vi "Request State Store.vi"(5 "arguments digest":string, 6 "name":string, 7 "method":string, 8 "error in":errorcluster, 9 "state":string, 10 "token":string, 11 "action":enum16{"store", "take", "clear"}(ring)) -> (0 "error out":errorcluster, 1 "entry":T1, 2 "found?":bool, 3 "new token":string)   [LabVIEW 2020, in "MCP Server.lvlib"]
doc: "Keeps the server-side state of multi round-trip requests (MCP 2026-07-28, requestState) and hands out the opaque tokens that stand for it. A functional global: the entries live in uninitialized shift registers of this non-reentrant VI, so every caller in the application instance sees the same store.\n\nWHY: a tool that asks several questions in several rounds (Ask User.vi) needs the answers of the earlier rounds, but the client sends back only the answers to the latest inputRequests. So the server keeps the earlier answers here and gives the client only a random token as requestState. The client never holds content it could tamper with; an unknown, expired or mis-bound token is simply not found.\n\naction:\n- store: keeps {token, state, method, name, arguments digest, created} and returns the new token. The token is \"mcp-rs-\" followed by 32 hex characters, the first half (16 bytes) of the SHA-256 (SHA-256 Byte Array Checksum.vi of NI's Message Digest API) of four random numbers, the tick count, a running counter and the state text.\n- take: looks the token up. found? is TRUE and entry holds the stored entry when it is known and not expired. Entries are NOT removed by take: a client may legitimately send the same round again after a network failure.\n- clear: forgets every entry.\n\nEvery call first drops the entries older than 10 minutes (600000 ms by Tick Count), and store keeps at most the 64 newest entries.\n\nUsed by Resolve Request State.vi (take) and Input Required Response.vi (store). error in is passed through unchanged; the store works whatever error in carries, and has no errors of its own."
uses:
  MCP Server.lvlib
  <vilib>/security/Message Digest/API/NI_Message Digest API.lvlib
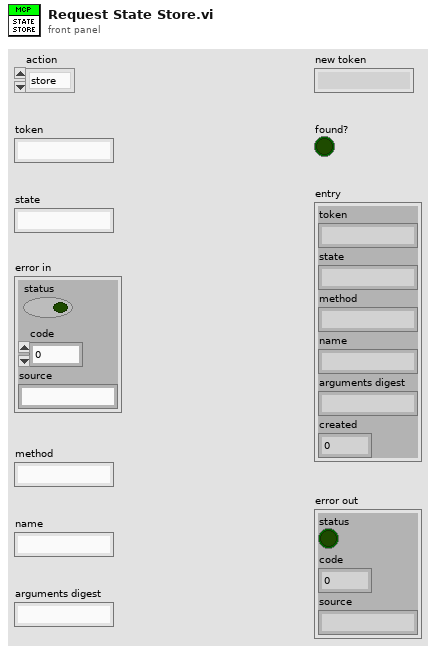
[diagram p1: front panel]
types:
  T1 = cluster{"token":string, "state":string, "method":string, "name":string, "arguments digest":string, "created":u32}
  T2 = cluster{"token":string, "state":string, "method":string, "name":string, "arguments digest":string, "created":u32}[]
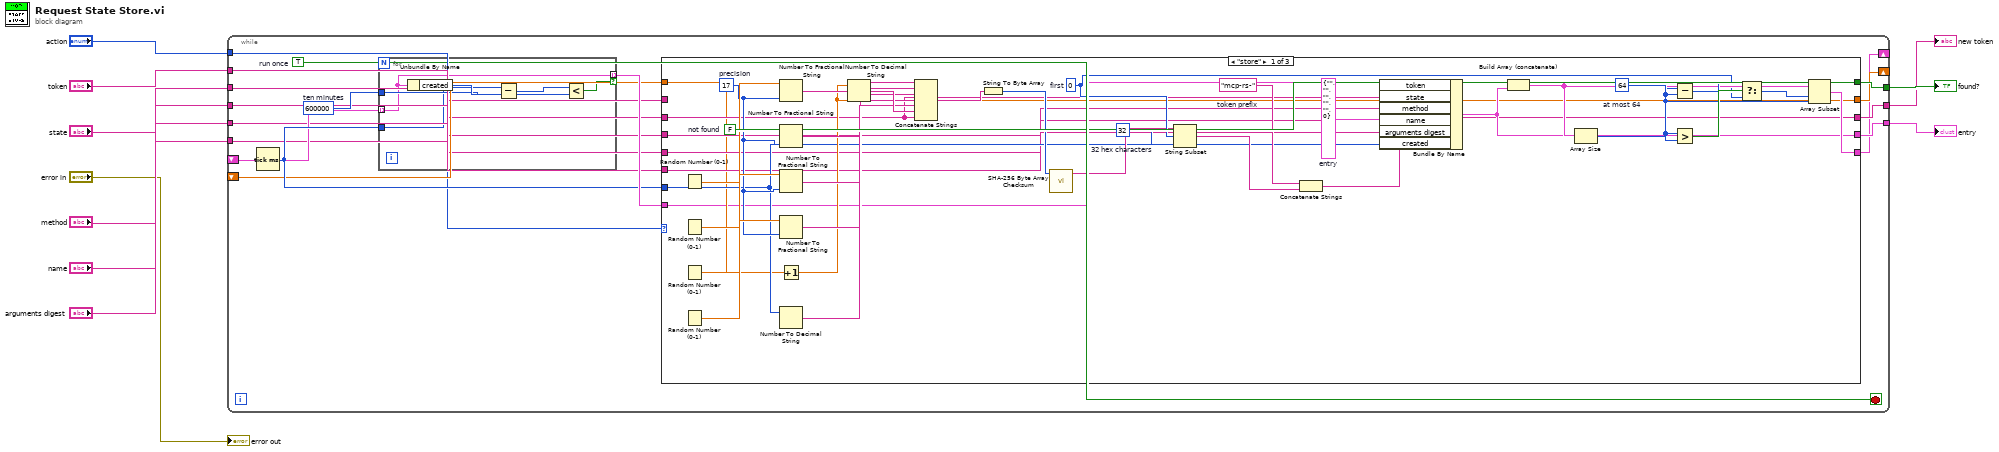
[diagram p0: block diagram]
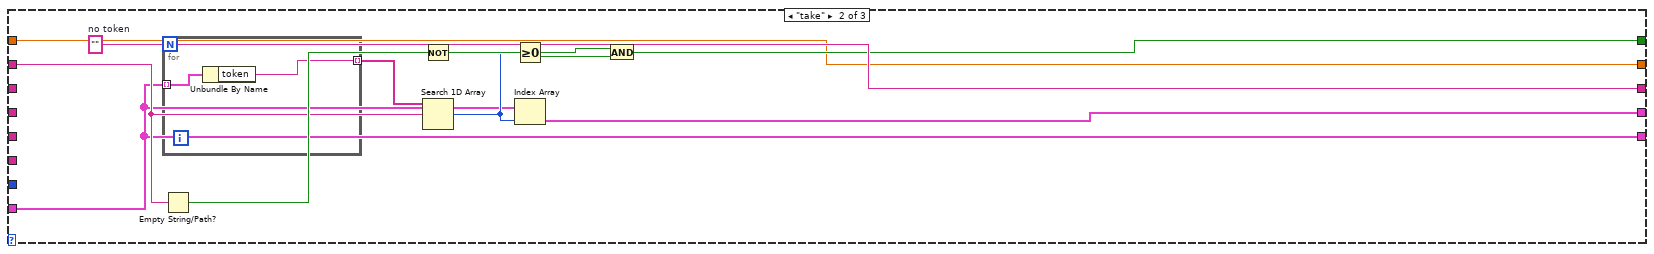
[diagram p2: hidden frame]
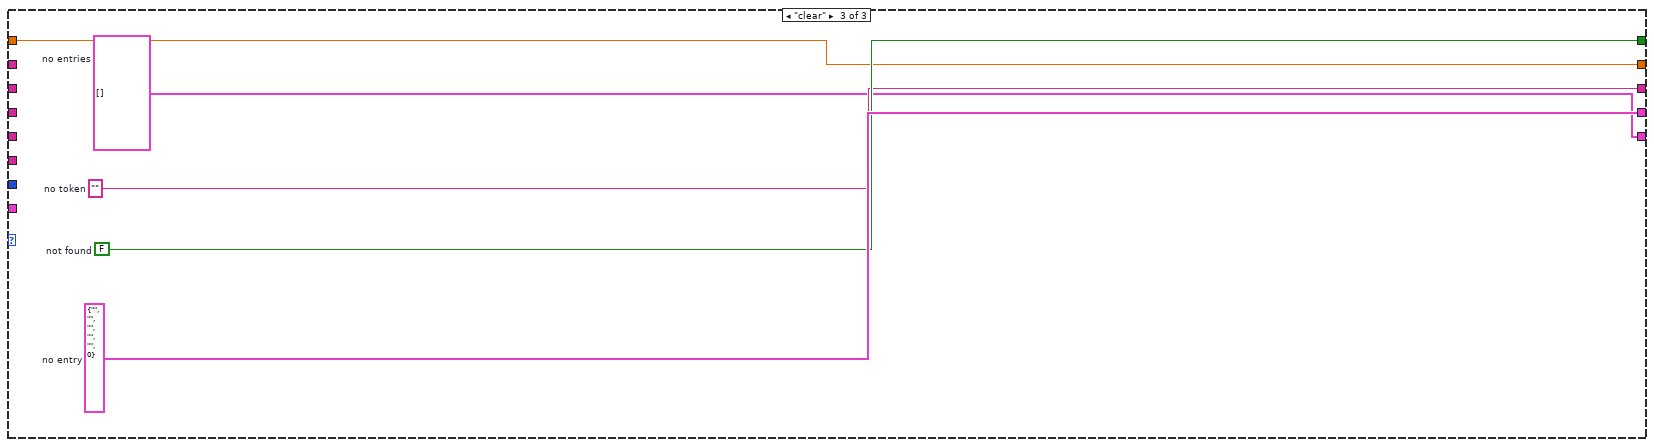
[diagram p3: hidden frame]
diagram:
  n1 = while {
    tunnel: "action" -> [w12]
    tunnel: "token" -> [w13]
    tunnel: "state" -> [w14]
    tunnel: "method" -> [w15]
    tunnel: "name" -> [w16]
    tunnel: "arguments digest" -> [w17]
    shift-right: [w19] -> _
    shift-left: _ -> [w18]
    shift-right: [w21] -> _
    shift-left: _ -> [w20]
    tunnel: [w26] -> w9
    tunnel: [w25] -> w8
    tunnel: [w27] -> w10
    stop <- w11 stop-if-true
    w23 = u32 600000  # ten minutes
    w11 = TRUE  # run once
    n2 = Tick Count (ms)() -> (millisecond timer value=w22:u32)
    n3 = for {
      tunnel: w23 -> [w85]
      tunnel: w18 -> [w83] mode=indexing
      tunnel: w22 -> [w84]
      tunnel: [w83] -> w24 mode=indexing if=w88
      n4 = Unbundle By Name(w83) -> ("created"=w86:u32)
      n5 = Subtract(x=w84, y=w86) -> (x-y=w87:u32)
      n6 = Less?(x=w87, y=w85) -> (x < y?=w88:bool)
    }
    n7 = case shown="\"store\"" w12 {
      tunnel: [w64 w73 w81] -> w26
      tunnel: w20 -> [w29 w66 w78]
      tunnel: w13 -> [_ w67 _]
      tunnel: w14 -> [w30 _ _]
      tunnel: w15 -> [w31 _ _]
      tunnel: w16 -> [w32 _ _]
      tunnel: w17 -> [w33 _ _]
      tunnel: w22 -> [w34 _ _]
      tunnel: w24 -> [w28 w65 _]
      tunnel: [w35 w66 w78] -> w21
      tunnel: [w54 w75 w80] -> w25
      tunnel: [w56 w74 w82] -> w27
      tunnel: [w63 w65 w79] -> w19
      frame "store" {
        w64 = FALSE  # not found
        w59 = 64  # at most 64
        w55 = T1 {"token"="", "state"="", "method"="", "name"="", "arguments digest"="", "created"=0}  # entry
        w53 = "mcp-rs-"  # token prefix
        w51 = 32  # 32 hex characters
        w50 = 0  # first
        w36 = 17  # precision
        n8 = Random Number (0-1)() -> (number: 0 to 1=w37:dbl)
        n9 = Random Number (0-1)() -> (number: 0 to 1=w39:dbl)
        n10 = Random Number (0-1)() -> (number: 0 to 1=w41:dbl)
        n11 = Random Number (0-1)() -> (number: 0 to 1=w43:dbl)
        n12 = Number To Fractional String(number=w37, precision (6)=w36) -> (F-format string=w38:string)  [unwired: 2 out]
        n13 = Number To Fractional String(number=w39, precision (6)=w36) -> (F-format string=w40:string)  [unwired: 2 out]
        n14 = Number To Fractional String(number=w41, precision (6)=w36) -> (F-format string=w42:string)  [unwired: 2 out]
        n15 = Number To Fractional String(number=w43, precision (6)=w36) -> (F-format string=w44:string)  [unwired: 2 out]
        n16 = Increment(x=w29) -> (x+1=w35:dbl)
        n17 = Number To Decimal String(number=w34) -> (decimal integer string=w45:string)  [unwired: 1 in]
        n18 = Number To Decimal String(number=w35) -> (decimal integer string=w46:string)  [unwired: 1 in]
        n19 = Concatenate Strings(w38, w40, w42, w44, w45, w46, w30) -> (w47:string)
        n20 = String To Byte Array(string=w47) -> (unsigned byte array=w48:u8[])
        n21 = call <vilib>:"SHA-256 Byte Array Checksum.vi"("buffer"=w48) -> ("digest"=w49:string)  [unwired: 10 in]
        n22 = String Subset(string=w49, offset (0)=w50, length (rest)=w51) -> (substring=w52:string)
        n23 = Concatenate Strings(w53, w52) -> (w54:string)
        n24 = Bundle By Name(cluster=w55, "token"=w54, "state"=w30, "method"=w31, "name"=w32, "arguments digest"=w33, "created"=w34) -> (w56:T1)
        n25 = Build Array (concatenate)(w28, w56) -> (w57:T2)
        n26 = Array Size(array=w57) -> (size(s)=w58:i32)
        n27 = Subtract(x=w58, y=w59) -> (x-y=w60:i32)
        n28 = Greater?(x=w58, y=w59) -> (0:w61:bool)
        n29 = Select(t=w60, s=w61, f=w50) -> (s? t:f=w62:i32)
        n30 = Array Subset(array=w57, index=w62, length=w59) -> (w63:T2)
      }
      frame "take" {
        w75 = ""  # no token
        n31 = for {
          tunnel: w65 -> [w76] mode=indexing
          tunnel: [w77] -> w68 mode=indexing
          n32 = Unbundle By Name(w76) -> ("token"=w77:string)
        }
        n33 = Empty String/Path?(string/path=w67) -> (empty?=w71:bool)
        n34 = Not(x=w71) -> (.not. x?=w72:bool)
        n35 = Search 1D Array(1D array=w68, element=w67) -> (index of element=w69:i32)  [unwired: 1 in]
        n36 = Greater Or Equal To 0?(x=w69) -> (x >= 0?=w70:bool)
        n37 = Index Array(array=w65, index=w69) -> (element=w74:T1)
        n38 = And(x=w70, y=w72) -> (x .and. y?=w73:bool)
      }
      frame "clear" {
        w82 = T1 {"token"="", "state"="", "method"="", "name"="", "arguments digest"="", "created"=0}  # no entry
        w81 = FALSE  # not found
        w80 = ""  # no token
        w79 = T2 []  # no entries
      }
    }
  }
  "new token" <- w8
  "found?" <- w9
  "entry" <- w10
  "error out" <- "error in"
